vi "lane_color.vi"(9 "Rx":dbl, 10 "Lx":dbl, 11 "image in":T1) -> (2 "R_color":string, 3 "L_color":string)   [LabVIEW 2024]
uses:
  <vilib>/vision/Image Controls.llb/IMAQ Image.ctl
  <vilib>/vision/NI_Vision_Development_Module.lvlib
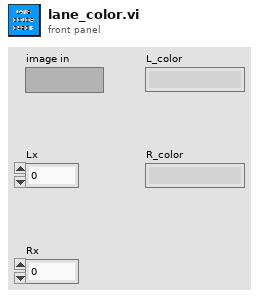
[diagram p1: front panel]
types:
  T1 = typedef "IMAQ Image.ctl" = refnum<image>
  T2 = cluster{"Red (or Hue) value":u8, "Green (or Sat) value":u8, "Blue (or Light or Val) value":u8}
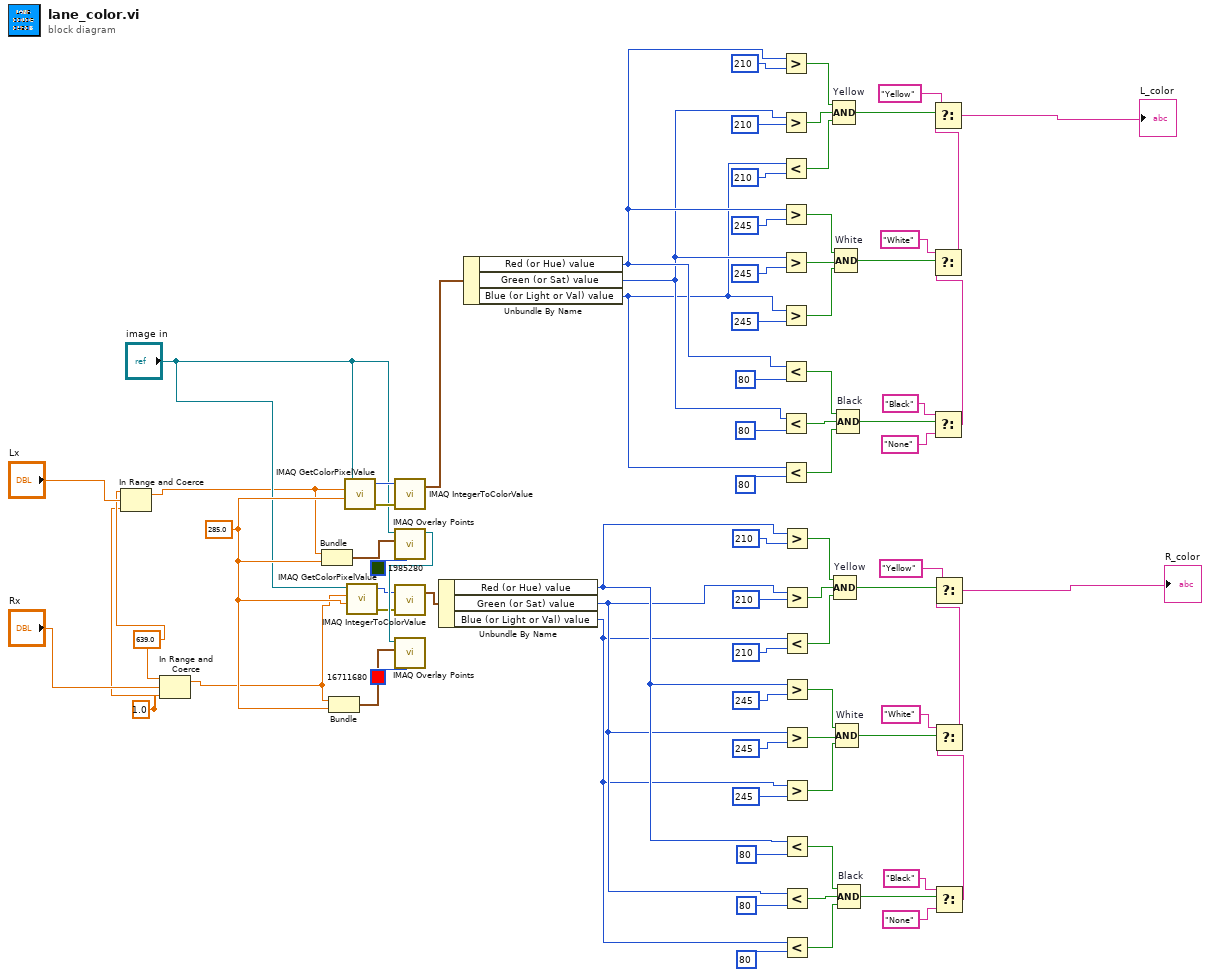
[diagram p0: block diagram]
diagram:
  w1 = 1.0 ("lower limit")
  w2 = 639.0 ("upper limit")
  w81 = 285.0 ("Ly")
  n1 = In Range and Coerce(upper limit=w2, x="Lx", lower limit=w1) -> (coerced(x)=w3:dbl)  [unwired: 1 out]
  n2 = In Range and Coerce(upper limit=w2, x="Rx", lower limit=w1) -> (coerced(x)=w6:dbl)  [unwired: 1 out]
  n3 = Bundle("upper limit"=w3, "Ly"=w81) -> (w77:cluster{"upper limit":dbl, "Ly":dbl})  [unwired: 1 in]
  n4 = Bundle("upper limit"=w6, "Ly"=w81) -> (w78:cluster{"upper limit":dbl, "Ly":dbl})  [unwired: 1 in]
  n5 = call "IMAQ GetColorPixelValue"("Y Coordinate"=w81, "X Coordinate"=w3, "Image"="image in") -> ("error out"=w43:errorcluster, "Pixel Value (U32)"=w40:u32)  [unwired: 1 in, 1 out]
  n6 = call "IMAQ GetColorPixelValue"("Y Coordinate"=w81, "X Coordinate"=w6, "Image"="image in") -> ("error out"=w41:errorcluster, "Pixel Value (U32)"=w42:u32)  [unwired: 1 in, 1 out]
  n7 = call "IMAQ IntegerToColorValue"("error in (no error)"=w43, "U32 value"=w40) -> ("Color Value"=w39:T2)  [unwired: 3 in, 3 out]
  n8 = call "IMAQ Overlay Points"("Color"=u32 1985280, "Point"=w77, "Image"="image in") -> ("Image Out"=w76:T1)  [unwired: 7 in, 1 out]
  n9 = call "IMAQ IntegerToColorValue"("error in (no error)"=w41, "U32 value"=w42) -> ("Color Value"=w75:T2)  [unwired: 3 in, 3 out]
  n10 = call "IMAQ Overlay Points"("Color"=u32 16711680, "Point"=w78, "Image"=w76) -> ()  [unwired: 7 in, 2 out]
  n11 = Unbundle By Name(w75) -> ("Red (or Hue) value"=w62:u8, "Green (or Sat) value"=w58:u8, "Blue (or Light or Val) value"=w55:u8)
  n12 = Unbundle By Name(w39) -> ("Red (or Hue) value"=w26:u8, "Green (or Sat) value"=w22:u8, "Blue (or Light or Val) value"=w19:u8)
  n13 = Greater?(x=w26, y=u8 210) -> (0:w24:bool)
  n14 = Greater?(x=w22, y=u8 210) -> (0:w21:bool)
  n15 = Less?(x=w19, y=u8 210) -> (x < y?=w18:bool)
  n16 = Greater?(x=w26, y=u8 245) -> (0:w38:bool)
  n17 = Greater?(x=w22, y=u8 245) -> (0:w37:bool)
  n18 = Greater?(x=w19, y=u8 245) -> (0:w36:bool)
  n19 = Less?(x=w26, y=u8 80) -> (x < y?=w35:bool)
  n20 = Less?(x=w22, y=u8 80) -> (x < y?=w34:bool)
  n21 = Less?(x=w19, y=u8 80) -> (x < y?=w33:bool)
  n22 = Greater?(x=w62, y=u8 210) -> (0:w60:bool)
  n23 = Greater?(x=w58, y=u8 210) -> (0:w57:bool)
  n24 = Less?(x=w55, y=u8 210) -> (x < y?=w54:bool)
  n25 = Greater?(x=w62, y=u8 245) -> (0:w74:bool)
  n26 = Greater?(x=w58, y=u8 245) -> (0:w73:bool)
  n27 = Greater?(x=w55, y=u8 245) -> (0:w72:bool)
  n28 = Less?(x=w62, y=u8 80) -> (x < y?=w71:bool)
  n29 = Less?(x=w58, y=u8 80) -> (x < y?=w70:bool)
  n30 = Less?(x=w55, y=u8 80) -> (x < y?=w69:bool)
  n31 = Compound Arithmetic op=AND "Yellow"(w24, w21, w18) -> (w8:bool)
  n32 = Compound Arithmetic op=AND "Yellow"(w60, w57, w54) -> (w44:bool)
  n33 = Compound Arithmetic op=AND "White"(w38, w37, w36) -> (w16:bool)
  n34 = Compound Arithmetic op=AND "White"(w74, w73, w72) -> (w52:bool)
  n35 = Compound Arithmetic op=AND "Black"(w35, w34, w33) -> (w15:bool)
  n36 = Compound Arithmetic op=AND "Black"(w71, w70, w69) -> (w51:bool)
  n37 = Select(t="Black", s=w15, f="None") -> (s? t:f=w10:string)
  n38 = Select(t="White", s=w16, f=w10) -> (s? t:f=w11:string)
  n39 = Select(t="Yellow", s=w8, f=w11) -> (s? t:f=→"L_color":string)
  n40 = Select(t="Black", s=w51, f="None") -> (s? t:f=w46:string)
  n41 = Select(t="White", s=w52, f=w46) -> (s? t:f=w47:string)
  n42 = Select(t="Yellow", s=w44, f=w47) -> (s? t:f=→"R_color":string)
